vi "VIH Utility - FILE - Make Valid Filename.vi"(10 "comply to CHM (F)":bool, 11 "File Name in":string) -> (3 "File Name out":string)   [LabVIEW 2014]
doc: "::: VI Helpeks :::\nCopyright (c) 2000-2026 Konstantin Shifershteyn. All rights reserved."
panel:
  # "VI Helpeks\nCopyright (c) 2012-2026 Konstantin Shifershteyn"
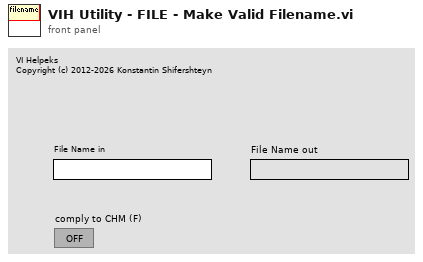
[diagram p1: front panel]
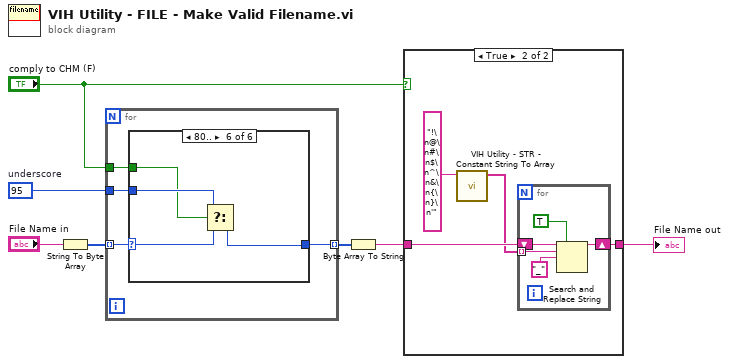
[diagram p0: block diagram]
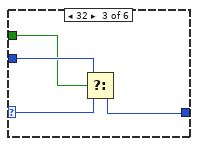
[diagram p5: hidden frame]
diagram:
  w7 = u8 95  # underscore
  n1 = String To Byte Array(string="File Name in") -> (unsigned byte array=w6:u8[])
  n2 = for {
    tunnel: w6 -> [w11] mode=indexing
    tunnel: [w10] -> w4 mode=indexing
    tunnel: w7 -> [w9]
    tunnel: "comply to CHM (F)" -> [w8]
    n3 = case shown="80.." w11 {
      selector: w11 -> [w12 _ w17 _ _ w23]
      tunnel: [w12 w13 w16 w18 w19 w22] -> w10
      tunnel: w9 -> [_ w13 w15 w18 w19 w21]
      tunnel: w8 -> [_ _ w14 _ _ w20]
      frame Default {
      }
      frame 0..31 {
      }
      frame 32 {
        n4 = Select(t=w15, s=w14, f=w17) -> (s? t:f=w16:u8)
      }
      frame 34, 42, 47 {
        # "\" * /"
      }
      frame 58..60, 62, 91..93, 124 {
        # ": ; < > [ \\ ] |"
      }
      frame 128.. {
        n5 = Select(t=w21, s=w20, f=w23) -> (s? t:f=w22:u8)
      }
    }
  }
  n6 = Byte Array To String(unsigned byte array=w4) -> (string=w3:string)
  n7 = case shown="True" "comply to CHM (F)" {
    tunnel: w3 -> [w24 w28]
    tunnel: [w24 w27] -> w2
    frame False {
    }
    frame True {
      n8 = call "VIH Utility - STR - Constant String To Array.vi"("String in"="!\n@\n#\n$\n^\n&\n{\n}\n'") -> ("Array out"=w25:string[])  [unwired: 10 in]
      n9 = for {
        shift-right: [w32] -> w27
        shift-left: w28 -> [w33]
        tunnel: w25 -> [w31] mode=indexing
        n10 = Search and Replace String(replace all?=TRUE, input string=w33, search string=w31, replace string="_") -> (result string=w32:string)  [unwired: 4 in, 3 out]
      }
    }
  }
  "File Name out" <- w2
